vi "Run Panel.vi"(7 "Set(F)":bool, 8 "error in (no error)":errorcluster, 10 "First Time(F)":bool, 11 "ChannelManagerUI in":refnum<class "ChannelManagerUI.lvclass">) -> (0 "error out":errorcluster, 1 "Changed?":bool, 2 "Channel":refnum<class "Channel.lvclass">, 3 "ChannelManagerUI out":refnum<class "ChannelManagerUI.lvclass">)   [LabVIEW 2021, in "Channel.lvlib" / "ChannelManagerUI.lvlib" / "ChannelManagerUI.lvclass"]
uses:
  ChannelManagerUI.lvclass
  Channel_class/Channel.lvclass
  Configuration_class/Configuration.lvclass
  ChannelManagerUI.lvclass/ChannelManagerUI.ctl
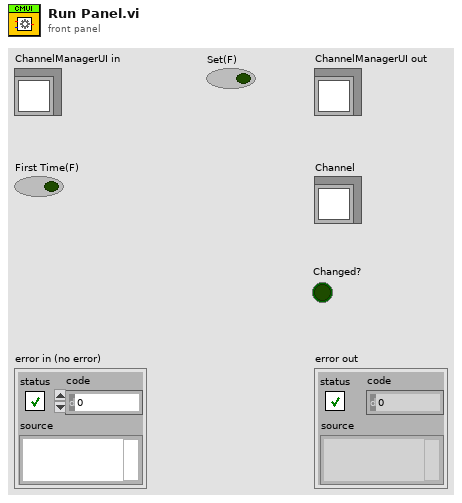
[diagram p1: front panel]
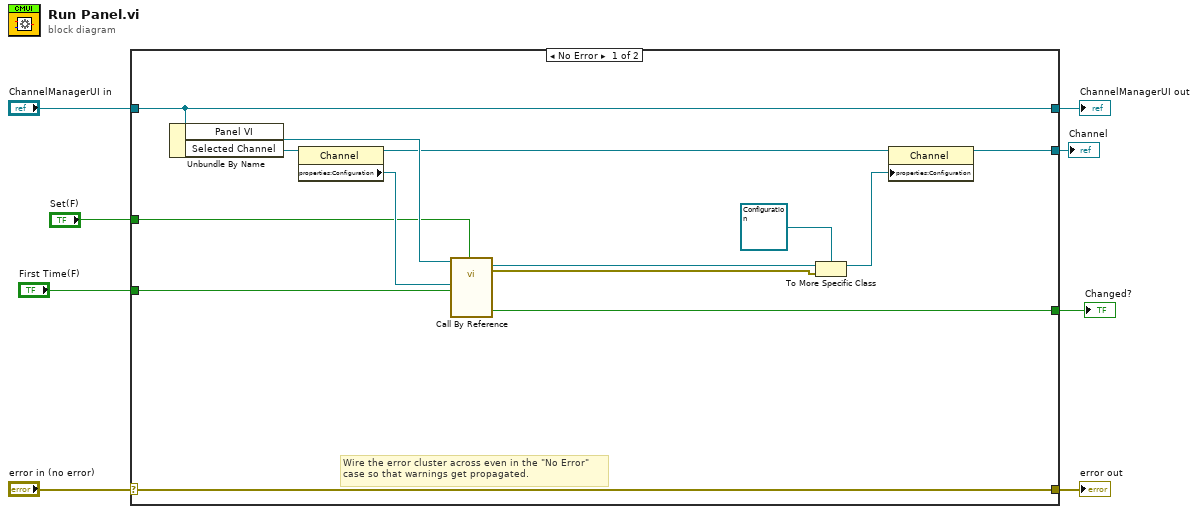
[diagram p0: block diagram]
diagram:
  n1 = case shown="No Error" "error in (no error)" {
    selector: "error in (no error)" -> [w22 w24]
    tunnel: [w22 w24] -> w7
    tunnel: [w17 w23] -> w5
    tunnel: "ChannelManagerUI in" -> [w17 w23]
    tunnel: [w12 _] -> w3
    tunnel: [w11 _] -> w4
    tunnel: "First Time(F)" -> [w10 _]
    tunnel: "Set(F)" -> [w9 _]
    frame No Error {
      # "Wire the error cluster across even in the \"No Error\"\ncase so that warnings get propagated."
      n2 = Unbundle By Name(w17) -> ("Panel VI"=w15:refnum<vi>, "Selected Channel"=w16:refnum<class "Channel.lvclass">)
      n3 = property class="Channel"(reference=w16) -> (reference out=w13:refnum<class "Channel.lvclass">, "properties:Configuration"=w14:refnum<class "Configuration.lvclass">)  [unwired: 1 in, 1 out]
      n4 = call-by-ref "?"(reference=w15, "Set(F)"=w9, "First Time(F)"=w10, "object in"=w14) -> (error out=w21:errorcluster, "Changed?"=w11:bool, "object out"=w20:refnum<class>)  [unwired: 7 in, 2 out]
      n5 = To More Specific Class(target class=refnum<class "Configuration.lvclass"> refnum ("Configuration"), reference=w20, error in=w21) -> (specific class reference=w19:refnum<class "Configuration.lvclass">)  [unwired: 1 out]
      n6 = property class="Channel"(reference=w13, "properties:Configuration"=w19) -> (reference out=w12:refnum<class "Channel.lvclass">)  [unwired: 1 in, 1 out]
    }
    frame Error {
    }
  }
  "error out" <- w7
  "ChannelManagerUI out" <- w5
  "Changed?" <- w4
  "Channel" <- w3
